vi "错误设备提示.vi"(6 "提示":bool=TRUE, 7 "Titre":string="遇到以下错误，将无法正常测试：", 9 "错误数组":errorcluster[](array[cluster]), 11 "设备列表":string[](array[string])) -> (0 "error out":errorcluster, 1 "out":string)   [LabVIEW 2025]
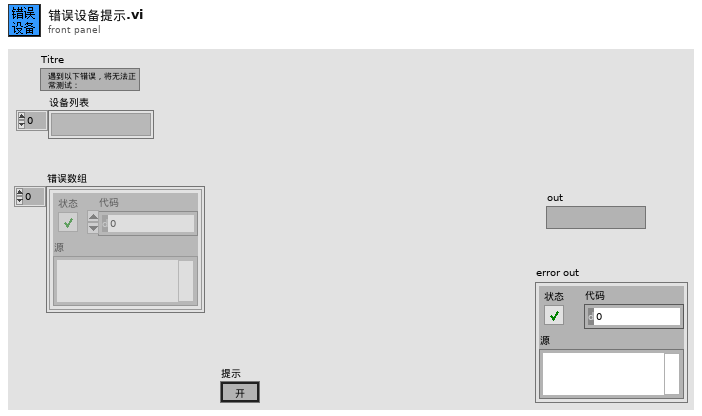
[diagram p1: front panel]
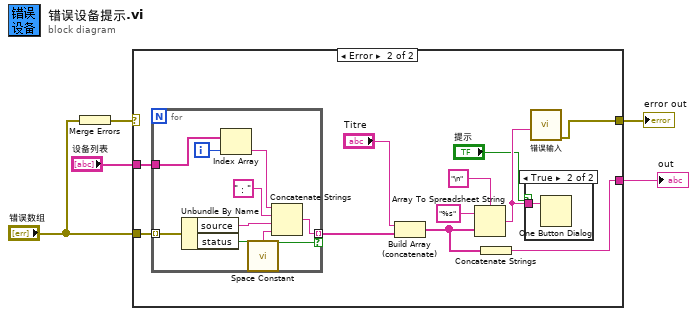
[diagram p0: block diagram]
diagram:
  n1 = Merge Errors("错误数组") -> (w5:errorcluster)
  n2 = case shown="Error" w5 {
    tunnel: "错误数组" -> [_ w16]
    tunnel: "设备列表" -> [_ w15]
    tunnel: [_ w11] -> w2
    tunnel: [_ w7] -> w1
    frame No Error {
    }
    frame Error {
      n3 = for {
        tunnel: w16 -> [w26] mode=indexing
        tunnel: w15 -> [w24]
        tunnel: [w23] -> w13 mode=indexing if=w19
        i -> [w25]
        n4 = Unbundle By Name(w26) -> ("source"=w20:string, "status"=w19:bool)
        n5 = Index Array(array=w24, index=w25) -> (element=w22:string)
        n6 = call <vilib>:"Space Constant.vi"() -> ("String"=w18:string)
        n7 = Concatenate Strings(w22, "：" ("字符串"), w20, w18) -> (w23:string)
      }
      n8 = Build Array (concatenate)("Titre", w13) -> (w8:string[])
      n9 = Array To Spreadsheet String(delimiter (Tab)="\n" ("分隔符(Tab)"), array=w8, 3:"%s" ("格式字符串")) -> (spreadsheet string=w9:string)
      n10 = Concatenate Strings(w8) -> (w7:string)
      n11 = case shown="True" "提示" {
        tunnel: w9 -> [_ w17]
        frame False {
        }
        frame True {
          n12 = One Button Dialog(message=w17) -> ()  [unwired: 1 in, 1 out]
        }
      }
      n13 = call "错误输入.vi"("source"=w9) -> ("error out"=w11:errorcluster)  [unwired: 10 in]
    }
  }
  "error out" <- w2
  "out" <- w1
